vi "test modern tools list.vi"(8 "error in (no error)":errorcluster) -> (0 "error out":errorcluster, 3 "body":string)   [LabVIEW 2020, in "MCP Server tests.lvlib"]
doc: "A request whose params._meta carries io.modelcontextprotocol/protocolVersion is answered in the MCP 2026-07-28 (modern) form: tools/list gets resultType complete, the caching hints ttlMs 60000 and cacheScope public, and _meta io.modelcontextprotocol/serverInfo. The same request without _meta is a legacy request and is answered exactly as before, without any of these fields. The requests are sent with the LabVIEW HTTP Client directly."
uses:
  MCP Server tests.lvlib
  <vilib>/JDP Science/JSONtext/Next JSON Value.vi
  <vilib>/JDP Science/JSONtext/String Subset.vi
  <vilib>/JDP Science/JSONtext/Parsing/Advance past next JSON Value (inlined COPY).vi
  <vilib>/JDP Science/JSONtext/Parsing/Advance past whitespace.vi
  <vilib>/JDP Science/JSONtext/Parsing/Advance past String.vi
  <vilib>/JDP Science/JSONtext/Parsing/Advance past Number.vi
  <vilib>/JDP Science/JSONtext/Parsing/Advance past Line Ending.vi
  <vilib>/JDP Science/JSONtext/Parsing/Parse Full Path or Item Name.vi
  <vilib>/JDP Science/JSONtext/Parsing/Advance past Array.vi
  <vilib>/JDP Science/JSONtext/Parsing/Advance past Object.vi
  <vilib>/JDP Science/JSONtext/support/Error Cluster From Code.vi
  <vilib>/JDP Science/JSONtext/Offset/Find Item Locations by Path.vi
  <vilib>/addons/_JKI Toolkits/Caraya/classes/Test/Test.lvclass
  <vilib>/JDP Science/JSONtext/JSONtext.lvlib
  <vilib>/addons/_JKI Toolkits/Caraya/classes/Assert/Assert.lvclass
panel:
  out "lookup error":errorcluster
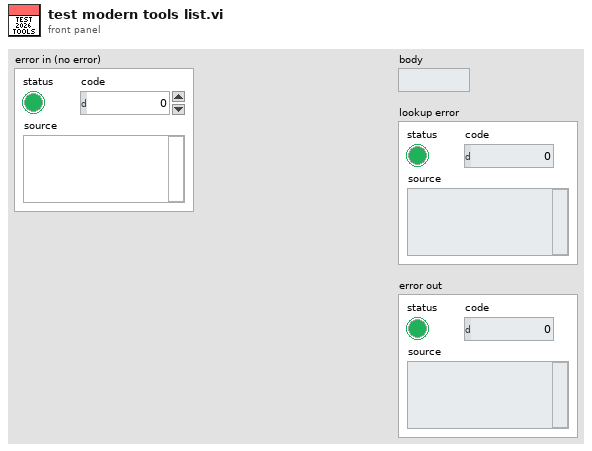
[diagram p1: front panel]
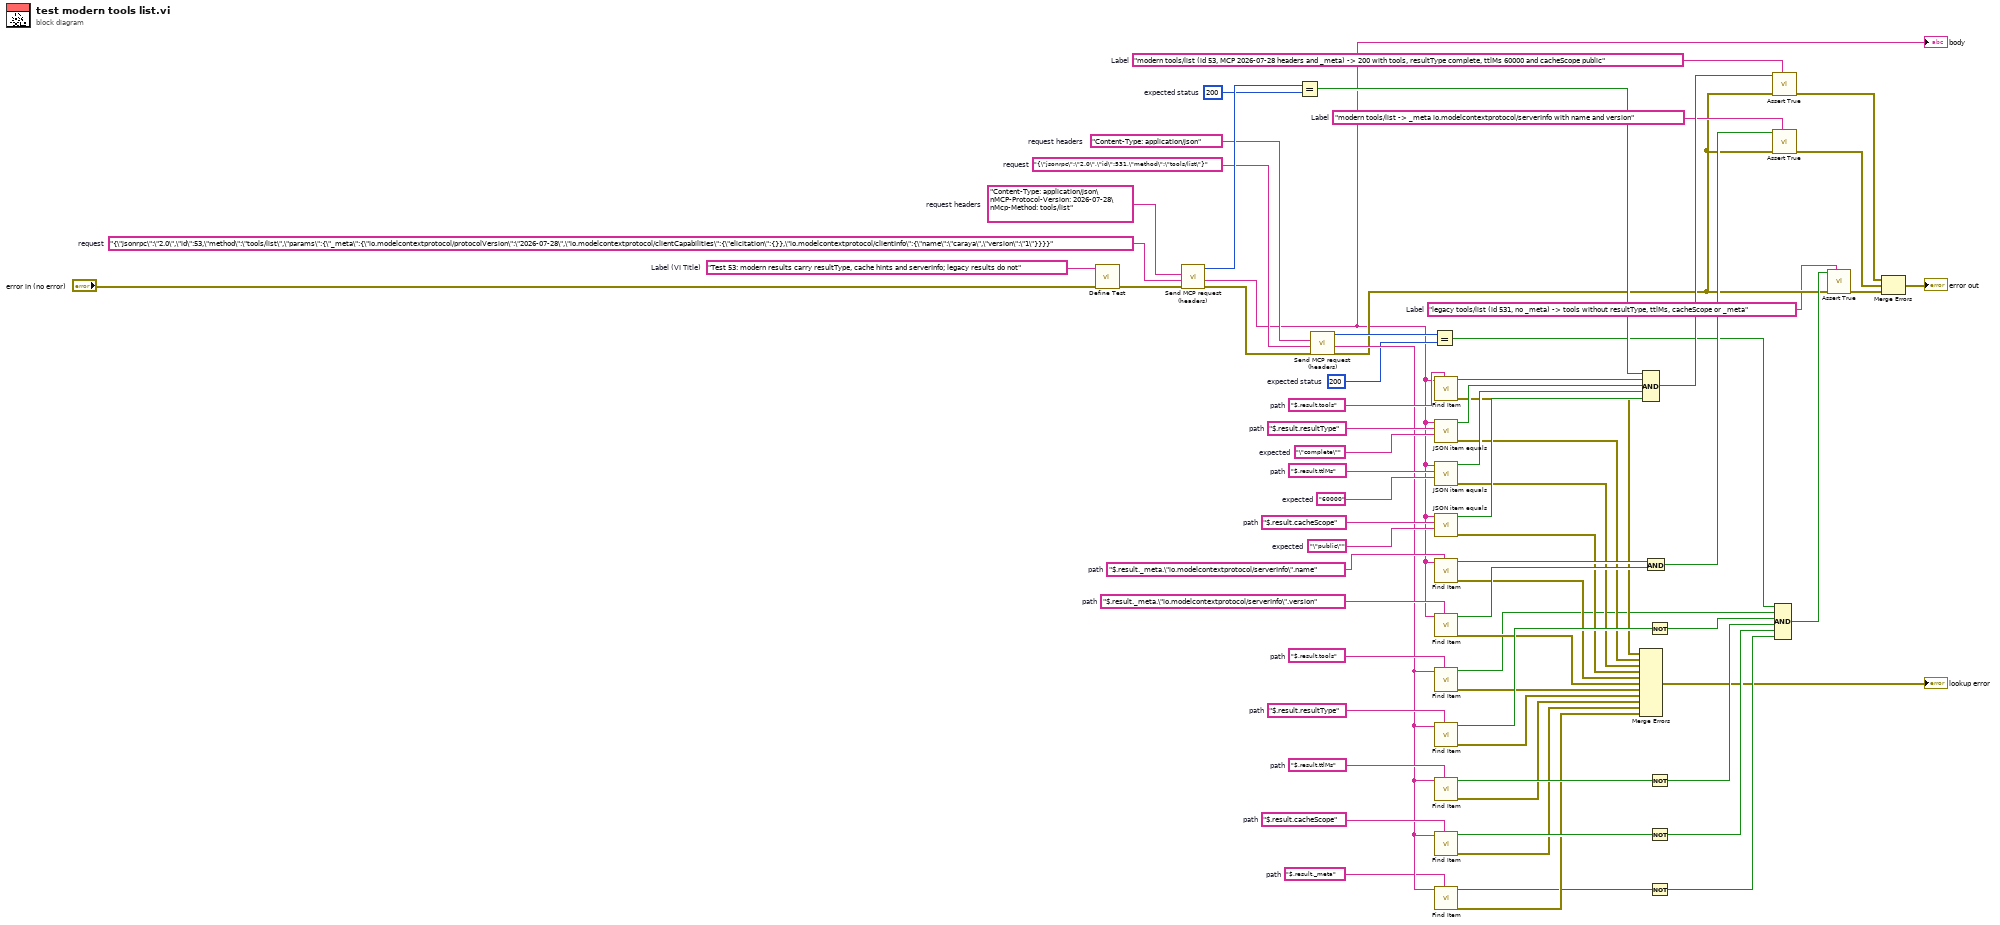
[diagram p0: block diagram]
diagram:
  w45 = "Content-Type: application/json"  # request headers
  w66 = "Content-Type: application/json\nMCP-Protocol-Version: 2026-07-28\nMcp-Method: tools/list"  # request headers
  w7 = "legacy tools/list (id 531, no _meta) -> tools without resultType, ttlMs, cacheScope or _meta"  # Label
  w18 = "modern tools/list -> _meta io.modelcontextprotocol/serverInfo with name and version"  # Label
  w20 = "modern tools/list (id 53, MCP 2026-07-28 headers and _meta) -> 200 with tools, resultType complete, ttlMs 60000 and cacheScope public"  # Label
  w37 = "$.result._meta"  # path
  w39 = "$.result.cacheScope"  # path
  w40 = "$.result.ttlMs"  # path
  w41 = "$.result.resultType"  # path
  w42 = "$.result.tools"  # path
  w16 = 200  # expected status
  w61 = "$.result._meta.\"io.modelcontextprotocol/serverInfo\".version"  # path
  w62 = "$.result._meta.\"io.modelcontextprotocol/serverInfo\".name"  # path
  w55 = "\"public\""  # expected
  w56 = "$.result.cacheScope"  # path
  w57 = "60000"  # expected
  w58 = "$.result.ttlMs"  # path
  w59 = "\"complete\""  # expected
  w60 = "$.result.resultType"  # path
  w63 = "$.result.tools"  # path
  w51 = 200  # expected status
  w44 = "{\"jsonrpc\":\"2.0\",\"id\":531,\"method\":\"tools/list\"}"  # request
  w65 = "{\"jsonrpc\":\"2.0\",\"id\":53,\"method\":\"tools/list\",\"params\":{\"_meta\":{\"io.modelcontextprotocol/protocolVersion\":\"2026-07-28\",\"io.modelcontextprotocol/clientCapabilities\":{\"elicitation\":{}},\"io.modelcontextprotocol/clientInfo\":{\"name\":\"caraya\",\"version\":\"1\"}}}}"  # request
  w68 = "Test 53: modern results carry resultType, cache hints and serverInfo; legacy results do not"  # Label (VI Title)
  n1 = call <vilib>:"Define Test.vi"("error in (no error)"="error in (no error)", "Label (VI Title)"=w68) -> ("error out"=w64:errorcluster)  [unwired: 8 in, 1 out]
  n2 = call "Send MCP request (headers).vi"("error in (no error)"=w64, "request"=w65, "request headers"=w66) -> ("error out"=w43:errorcluster, "response"=w3:string, "status code"=w52:i32)  [unwired: 5 in, 1 out]
  "body" <- w3
  n3 = Equal?(x=w52, y=w51) -> (x = y?=w50:bool)
  n4 = call "Send MCP request (headers).vi"("error in (no error)"=w43, "request"=w44, "request headers"=w45) -> ("error out"=w8:errorcluster, "response"=w38:string, "status code"=w17:i32)  [unwired: 5 in, 1 out]
  n5 = Equal?(x=w17, y=w16) -> (x = y?=w15:bool)
  n6 = call <vilib>:"Find Item.vi"("$Path or Item Name"=w63, "JSON"=w3) -> ("error out"=w33:errorcluster, "Found"=w49:bool)  [unwired: 6 in, 2 out]
  n7 = call "JSON item equals.vi"("expected"=w59, "path"=w60, "JSON"=w3) -> ("error out"=w32:errorcluster, "equal?"=w48:bool)  [unwired: 6 in, 1 out]
  n8 = call "JSON item equals.vi"("expected"=w57, "path"=w58, "JSON"=w3) -> ("error out"=w31:errorcluster, "equal?"=w47:bool)  [unwired: 6 in, 1 out]
  n9 = call "JSON item equals.vi"("expected"=w55, "path"=w56, "JSON"=w3) -> ("error out"=w30:errorcluster, "equal?"=w46:bool)  [unwired: 6 in, 1 out]
  n10 = call <vilib>:"Find Item.vi"("$Path or Item Name"=w62, "JSON"=w3) -> ("error out"=w29:errorcluster, "Found"=w54:bool)  [unwired: 6 in, 2 out]
  n11 = call <vilib>:"Find Item.vi"("$Path or Item Name"=w61, "JSON"=w3) -> ("error out"=w28:errorcluster, "Found"=w53:bool)  [unwired: 6 in, 2 out]
  n12 = call <vilib>:"Find Item.vi"("$Path or Item Name"=w42, "JSON"=w38) -> ("error out"=w27:errorcluster, "Found"=w14:bool)  [unwired: 6 in, 2 out]
  n13 = call <vilib>:"Find Item.vi"("$Path or Item Name"=w41, "JSON"=w38) -> ("error out"=w26:errorcluster, "Found"=w36:bool)  [unwired: 6 in, 2 out]
  n14 = call <vilib>:"Find Item.vi"("$Path or Item Name"=w40, "JSON"=w38) -> ("error out"=w25:errorcluster, "Found"=w35:bool)  [unwired: 6 in, 2 out]
  n15 = call <vilib>:"Find Item.vi"("$Path or Item Name"=w39, "JSON"=w38) -> ("error out"=w24:errorcluster, "Found"=w34:bool)  [unwired: 6 in, 2 out]
  n16 = call <vilib>:"Find Item.vi"("$Path or Item Name"=w37, "JSON"=w38) -> ("error out"=w23:errorcluster, "Found"=w22:bool)  [unwired: 6 in, 2 out]
  n17 = Merge Errors(w33, w32, w31, w30, w29, w28, w27, w26, w25, w24, w23) -> (→"lookup error":errorcluster)
  n18 = Compound Arithmetic op=AND(w50, w49, w48, w47, w46) -> (w21:bool)
  n19 = Compound Arithmetic op=AND(w54, w53) -> (w19:bool)
  n20 = Not(x=w36) -> (.not. x?=w13:bool)
  n21 = Not(x=w35) -> (.not. x?=w12:bool)
  n22 = Not(x=w34) -> (.not. x?=w11:bool)
  n23 = Not(x=w22) -> (.not. x?=w10:bool)
  n24 = call <vilib>:"Assert True.vi"("Label"=w20, "error in (no error)"=w8, "True?"=w21) -> ("error out"=w6:errorcluster)  [unwired: 7 in, 1 out]
  n25 = call <vilib>:"Assert True.vi"("Label"=w18, "error in (no error)"=w8, "True?"=w19) -> ("error out"=w5:errorcluster)  [unwired: 7 in, 1 out]
  n26 = Compound Arithmetic op=AND(w15, w14, w13, w12, w11, w10) -> (w9:bool)
  n27 = call <vilib>:"Assert True.vi"("Label"=w7, "error in (no error)"=w8, "True?"=w9) -> ("error out"=w4:errorcluster)  [unwired: 7 in, 1 out]
  n28 = Merge Errors(w6, w5, w4) -> (→"error out":errorcluster)
